vi "Table for rader value.vi"(5 "N_sort_#":string[](array[string]), 6 "error in (no error)":errorcluster, 7 "P_sort_#":string[](array[string]), 8 "P_sort_[%]":string[](array[string]), 9 "N_sort_[%]":string[](array[string]), 10 "P_sort_B":string[](array[string]), 11 "N_sort_B":string[](array[string])) -> (2 "Mono Table Tag":string[](array[string]), 3 "Mono Table":string[][](table) caption="B Table", 4 "error out":errorcluster)   [LabVIEW 2018]
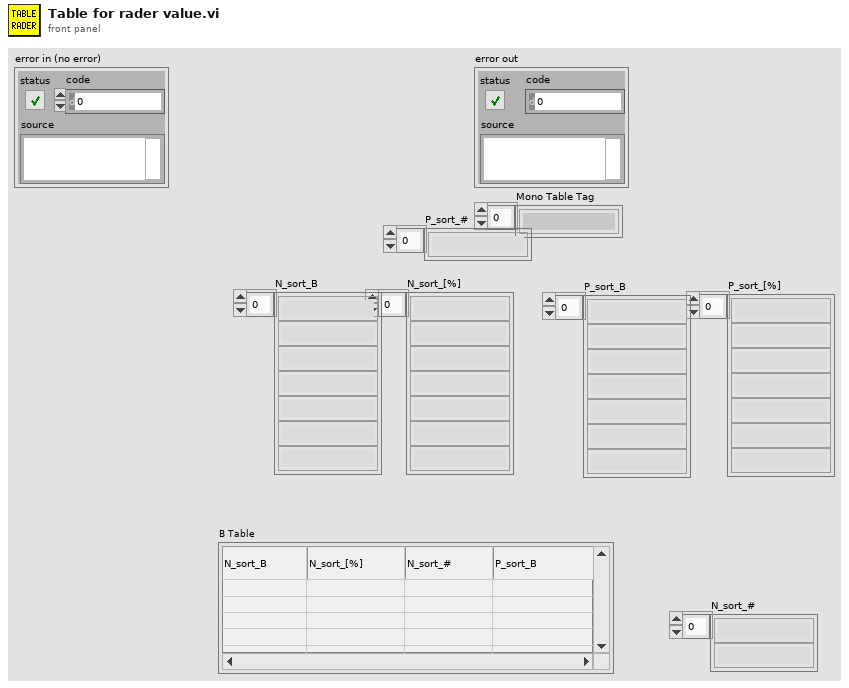
[diagram p1: front panel]
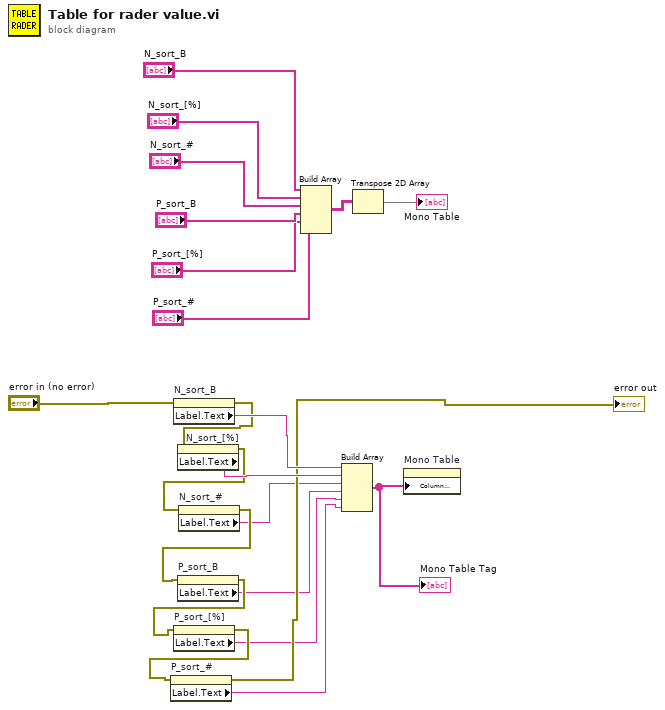
[diagram p0: block diagram]
diagram:
  n1 = property on="N_sort_B" class="Arr (strict)"(error in="error in (no error)") -> (error out=w14:errorcluster, "Label.Text"=w16:string)  [unwired: 1 in, 1 out]
  n2 = property on="N_sort_[%]" class="Arr (strict)"(error in=w14) -> (error out=w8:errorcluster, "Label.Text"=w15:string)  [unwired: 1 in, 1 out]
  n3 = property on="N_sort_#" class="Arr (strict)"(error in=w8) -> (error out=w7:errorcluster, "Label.Text"=w4:string)  [unwired: 1 in, 1 out]
  n4 = property on="P_sort_B" class="Arr (strict)"(error in=w7) -> (error out=w13:errorcluster, "Label.Text"=w3:string)  [unwired: 1 in, 1 out]
  n5 = property on="P_sort_[%]" class="Arr (strict)"(error in=w13) -> (error out=w6:errorcluster, "Label.Text"=w2:string)  [unwired: 1 in, 1 out]
  n6 = property on="P_sort_#" class="Arr (strict)"(error in=w6) -> (error out=→"error out":errorcluster, "Label.Text"=w1:string)  [unwired: 1 in, 1 out]
  n7 = Build Array("N_sort_B", "N_sort_[%]", "N_sort_#", "P_sort_B", "P_sort_[%]", "P_sort_#") -> (w20:string[][])
  n8 = Build Array(w16, w15, w4, w3, w2, w1) -> (w18:string[])
  "Mono Table Tag" <- w18
  n9 = Transpose 2D Array(2D array=w20) -> (transposed array=→"Mono Table":string[][])
  n10 = property on="Mono Table" class="Tbl (strict)"("Column Headers[]"=w18) -> ()  [unwired: 2 in, 2 out]
